vi "Decompose LabVIEW Object.vi"(8 "error in (no error)":errorcluster, 11 "LabVIEW Object":refnum<class>) -> (0 "error out":errorcluster, 1 "Class Names":string[](array[string]), 2 "Library Versions":T1(array[cluster]), 3 "Private Data Clusters":variant[](array[variant]))   [LabVIEW 2017, in "Composition.lvlib"]
doc: "Decomposes a LabVIEW Object into its private data clusters from oldest ancestor to last decendant (same order as in Probe Watch Window)."
uses:
  Composition.lvlib
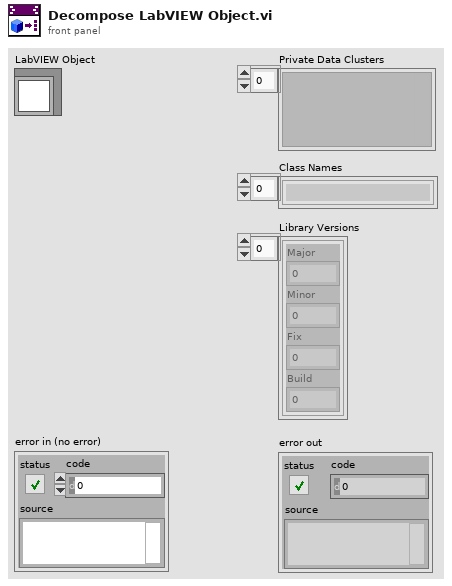
[diagram p1: front panel]
types:
  T1 = cluster{"Major":u16, "Minor":u16, "Fix":u16, "Build":u16}[]
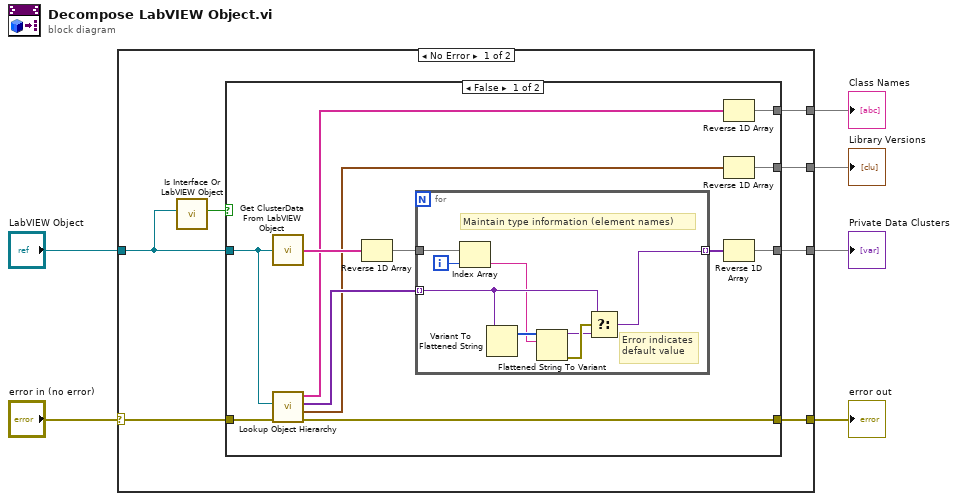
[diagram p0: block diagram]
diagram:
  n1 = case shown="No Error" "error in (no error)" {
    selector: "error in (no error)" -> [w10 w35]
    tunnel: [w13 _] -> w4
    tunnel: "LabVIEW Object" -> [w8 _]
    tunnel: [w9 w35] -> w3
    tunnel: [w12 _] -> w2
    tunnel: [w11 _] -> w1
    frame No Error {
      n2 = call "Is Interface Or LabVIEW Object.vi"("LabVIEW Object"=w8) -> ("Is Interface Or LabVIEW Object"=w7:bool)  [unwired: 10 in]
      n3 = case shown="False" w7 {
        tunnel: [w20 _] -> w13
        tunnel: w8 -> [w22 _]
        tunnel: [w17 _] -> w12
        tunnel: [w16 _] -> w11
        tunnel: w10 -> [w15 w34]
        tunnel: [w14 w34] -> w9
        frame False {
          n4 = call "Get ClusterData From LabVIEW Object.vi"("LabVIEW Object"=w22) -> ("Flattened Cluster Data"=w24:string[])
          n5 = call "Lookup Object Hierarchy.vi"("error in (no error)"=w15, "LabVIEW Object"=w22) -> ("error out"=w14:errorcluster, "Library Versions"=w18:T1, "Private Data Clusters"=w21:variant[], "Class Names"=w19:string[])  [unwired: 6 in]
          n6 = Reverse 1D Array(array=w24) -> (reversed array=w25:string[])
          n7 = for {
            tunnel: w25 -> [w29]
            tunnel: [w26] -> w23 mode=indexing
            tunnel: w21 -> [w30] mode=indexing
            i -> [w28]
            # "Error indicates\ndefault value"
            # "Maintain type information (element names)"
            n8 = Index Array(array=w29, index=w28) -> (element=w27:string)
            n9 = Variant To Flattened String(Variant=w30) -> (1:w33:i16[])  [unwired: 1 out]
            n10 = Flattened String To Variant(6:w27, 7:w33) -> (0:w32:errorcluster, 3:w31:variant)  [unwired: 1 in]
            n11 = Select(t=w30, s=w32, f=w31) -> (s? t:f=w26:variant)
          }
          n12 = Reverse 1D Array(array=w19) -> (reversed array=w17:string[])
          n13 = Reverse 1D Array(array=w18) -> (reversed array=w16:T1)
          n14 = Reverse 1D Array(array=w23) -> (reversed array=w20:variant[])
        }
        frame True {
          # "Ignore LabVIEW Object (mother of all objects in LV)"
        }
      }
    }
    frame Error {
    }
  }
  "Private Data Clusters" <- w4
  "error out" <- w3
  "Class Names" <- w2
  "Library Versions" <- w1
